vi "Is LVUnit Test.vi"(11 "ProjectItem Refnum":refnum<vi>) -> (2 "Is LVUnit Test":bool)   [LabVIEW 2017, in "LVUnit Test Discoverer.lvclass"]
uses:
  LVUnit Test Discoverer.lvclass
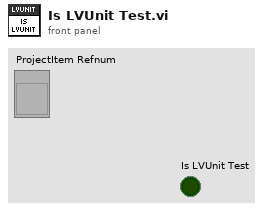
[diagram p1: front panel]
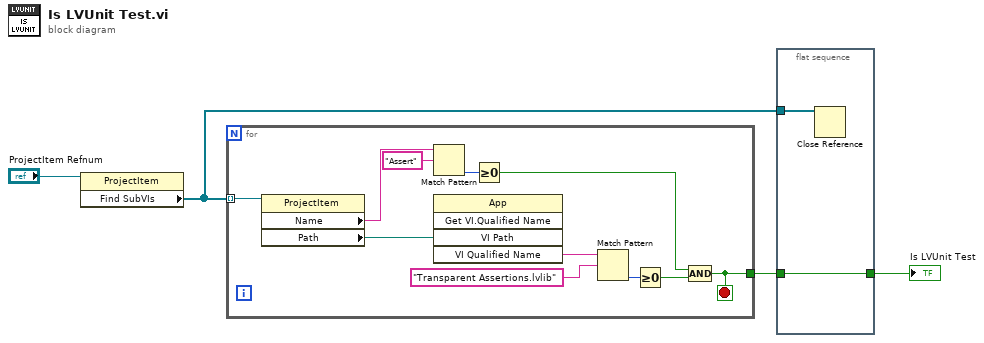
[diagram p0: block diagram]
diagram:
  n1 = property class="ProjectItem"(reference="ProjectItem Refnum") -> ("Find SubVIs"=w3:refnum<vi>[])  [unwired: 1 in, 2 out]
  n2 = for {
    tunnel: w3 -> [w15] mode=indexing
    tunnel: [w12] -> w1
    stop <- w12 stop-if-true
    n3 = property class="ProjectItem"(reference=w15) -> ("Name"=w11:string, "Path"=w14:path)  [unwired: 1 in, 2 out]
    n4 = Match Pattern(string=w11, regular expression="Assert") -> (offset past match=w9:i32)  [unwired: 1 in, 3 out]
    n5 = invoke class="App" method="Get VI.Qualified Name"("VI Path"=w14) -> ("VI Qualified Name"=w7:string)  [unwired: 4 in, 4 out]
    n6 = Greater Or Equal To 0?(x=w9) -> (x >= 0?=w8:bool)
    n7 = Match Pattern(string=w7, regular expression="Transparent Assertions.lvlib") -> (offset past match=w5:i32)  [unwired: 1 in, 3 out]
    n8 = Greater Or Equal To 0?(x=w5) -> (x >= 0?=w13:bool)
    n9 = Compound Arithmetic op=AND(w8, w13) -> (w12:bool)
  }
  n10 = flat-sequence {
    tunnel: w3 -> [w17]
    tunnel: [w16] -> w2
    tunnel: w1 -> [w16]
    frame #0 {
      n11 = Close Reference(reference=w17) -> ()  [unwired: 1 in, 1 out]
    }
  }
  "Is LVUnit Test" <- w2
